vi "Format EoL for CSV(Unicode).vi"(11 "base string":string) -> (3 "String out":string)   [LabVIEW 2019, in "Language Editor.lvlib"]
doc: "- - -\nCopyright (c) 2026, Merecs Engineering GmbH"
uses:
  Language Editor.lvlib
panel:
  # "Connector Pane"
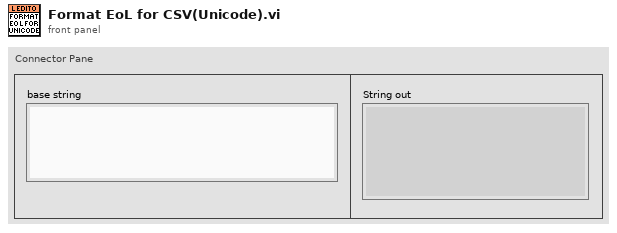
[diagram p1: front panel]
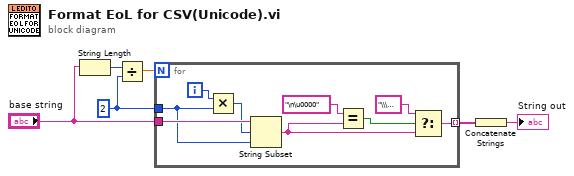
[diagram p0: block diagram]
diagram:
  w1 = 2 ("y")
  n1 = String Length(string="base string") -> (length=w6:i32)
  n2 = Divide(x=w6, y=w1) -> (x/y=w2:dbl)
  n3 = for {
    N: w2 -> [_]
    tunnel: "base string" -> [w15]
    tunnel: [w8] -> w4 mode=indexing
    tunnel: w1 -> [w12]
    i -> [w14]
    n4 = Multiply(x=w14, y=w12) -> (x*y=w13:i32)
    n5 = String Subset(string=w15, offset (0)=w13, length (rest)=w12) -> (substring=w9:string)
    n6 = Equal?(x="\n\u0000" ("search string"), y=w9) -> (x = y?=w10:bool)
    n7 = Select(t="\\\u0000n\u0000" ("search string"), s=w10, f=w9) -> (s? t:f=w8:string)
  }
  n8 = Concatenate Strings(w4) -> (→"String out":string)
